vi "Read Events.vi"(8 "error in (no error)":errorcluster, 11 "WebView2 Control in":refnum<class "WebView2 QControl.lvclass">=refnum) -> (0 "error out":errorcluster, 2 "Events":T1, 3 "WebView2 Control out":refnum<class "WebView2 QControl.lvclass">)   [LabVIEW 2020, in "WebView2 QControl.lvlib" / "WebView2 QControl.lvclass"]
uses:
  WebView2 QControl.lvclass
  WebView2 QControl.lvclass/WebView2 QControl.ctl
  Webview2 Lib/WebView2 Control Object/WebView2 Control.lvclass
  Webview2 Lib/WebView2 Control Object/Navigation Event Data.ctl
  Webview2 Lib/WebView2 Control Object/Source Changed Event Data.ctl
  Webview2 Lib/WebView2 Control Object/Navigation Start Event Data.ctl
  Webview2 Lib/WebView2 Control Object/Events.ctl
  Webview2 Lib/WebView2 Control Object/Web Message Received Event Data.ctl
  Webview2 Lib/WebView2 Event Filter Interface/WebView2 Event Filter Interface.lvclass
  E:/Labview/LV 2023/PPL/PPL Builder/Libs/LV-WebView2/Source/Libs/Microsoft.Web.WebView2.Core.dll
  Libs/Microsoft.Web.WebView2.Core.dll
  Webview2 Lib/WebView2 Control Object/New Window Event Data.ctl
  Webview2 Lib/WebView2 Control Object/Content Loading Event Data.ctl
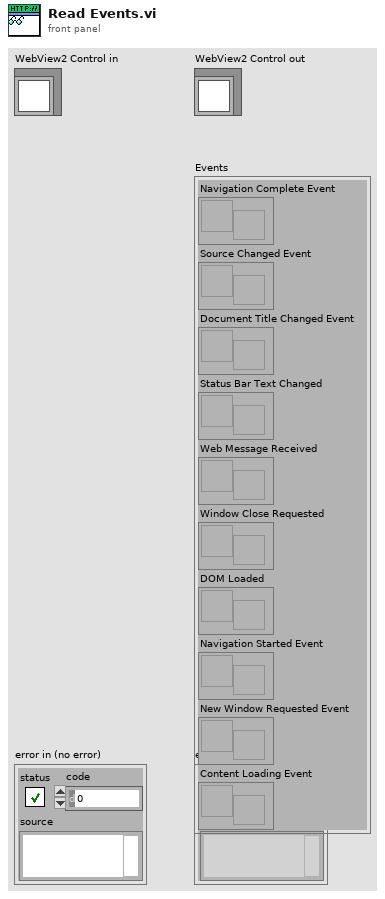
[diagram p1: front panel]
types:
  T1 = typedef "WebView2.lvlib/WebView2 Control.lvclass/Events.ctl" = cluster{"Navigation Complete Event":refnum<user-event>, "Source Changed Event":refnum<user-event>, "Document Title Changed Event":refnum<user-event>, "Status Bar Text Changed":refnum<user-event>, "Web Message Received":refnum<user-event>, "Window Close Requested":refnum<user-event>, "DOM Loaded":refnum<user-event>, "Navigation Started Event":refnum<user-event>, "New Window Requested Event":refnum<user-event>, "Content Loading Event":refnum<user-event>}
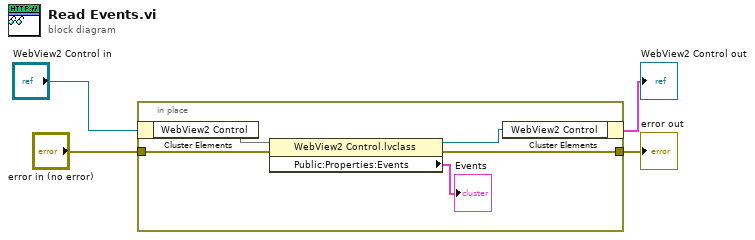
[diagram p0: block diagram]
diagram:
  n1 = in-place {
    in-place-border: "error in (no error)" -> [w9]
    in-place-border: [w8] -> w1
    n2 = in-place-cluster #1("WebView2 Control in") -> ("WebView2 Control"=w7)
    n3 = property class="WebView2 Control.lvclass"(reference=w7, error in=w9) -> (reference out=w6:refnum<class "WebView2 Control.lvclass">, error out=w8:errorcluster, "Public:Properties:Events"=→"Events":T1)
    n4 = in-place-cluster #1("WebView2 Control"=w6) -> (→"WebView2 Control out":cluster{})
  }
  "error out" <- w1
